vi "ModbusReadHD220.vi"(0 "Modbus master out 3":refnum<class "Modbus Master.lvclass">, 11 "error in (no error)":errorcluster caption="에러 입력(에러 없음)") -> (4 "Modbus master out":refnum<class "Modbus Master.lvclass">, 6 "24105":u16[](array[numeric]), 8 "20600":bool[](array[boolean]), 13 "21600(0)":bool[](array[boolean]), 14 "21600(1)":bool[](array[boolean]), 15 "error out":errorcluster caption="에러 출력")   [LabVIEW 2019]
uses:
  <vilib>/NI/Modbus Library/API/Master/Modbus Master.lvclass
panel:
  out "24019":u16[](array[numeric])
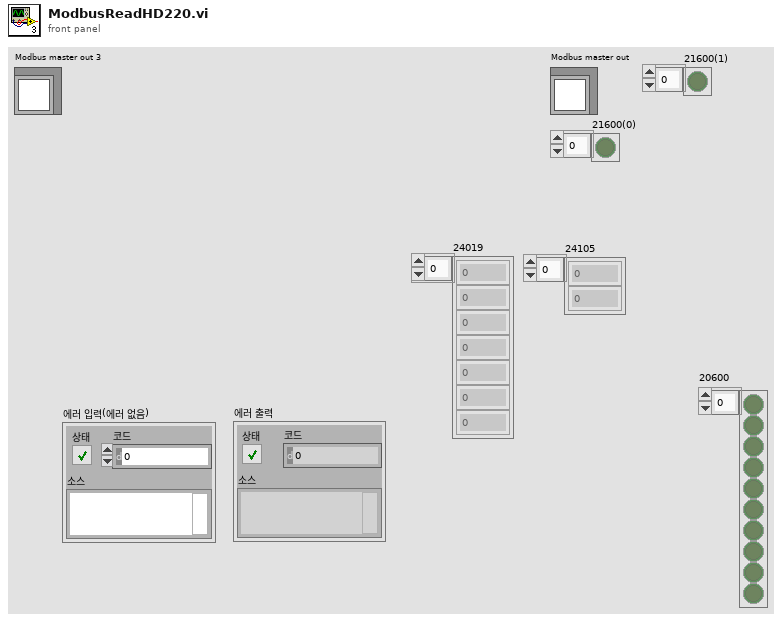
[diagram p1: front panel]
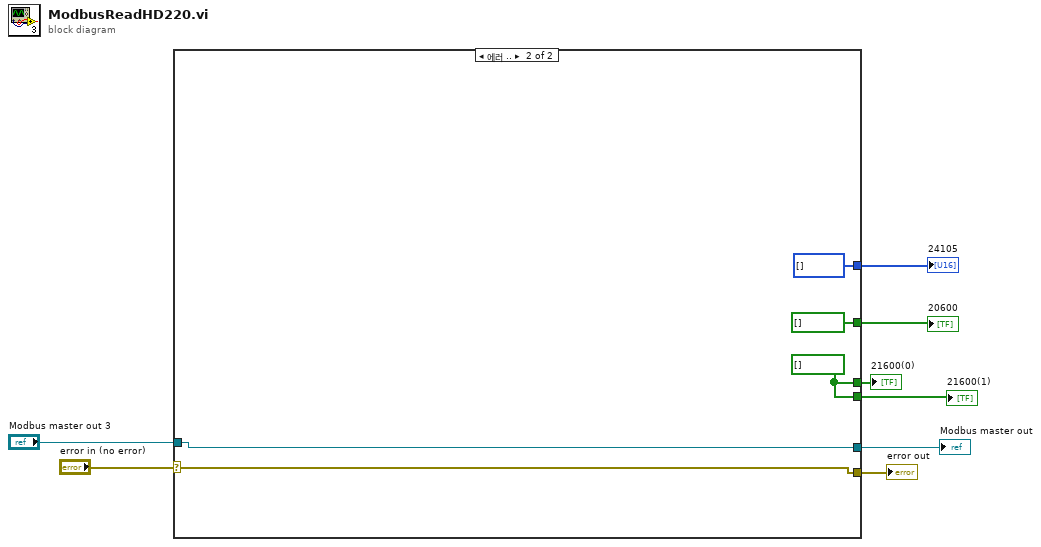
[diagram p0: block diagram]
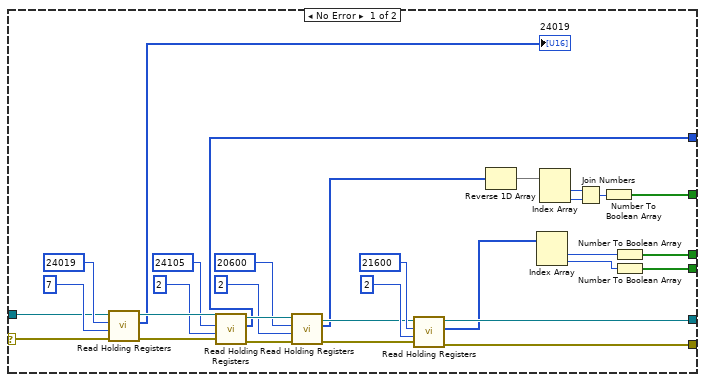
[diagram p2: hidden frame]
diagram:
  n1 = case shown="에러 .." "error in (no error)" {
    selector: "error in (no error)" -> [w37 w43]
    tunnel: "Modbus master out 3" -> [w32 w44]
    tunnel: [w23 w43] -> w6
    tunnel: [w22 w44] -> w5
    tunnel: [w15 bool[] [] ("Boolean array")] -> w4
    tunnel: [w14 u16[] [] ("register values")] -> w3
    tunnel: [w10 w40] -> w1
    tunnel: [w9 w40] -> w2
    frame No Error {
      n2 = call-dynamic "Read Holding Registers.vi"("error in"=w37, "number of inputs"=u16 7, "starting address"=u16 24019, "Modbus master in"=w32) -> ("error out"=w36:errorcluster, "register values"=→"24019":u16[], "Modbus master out"=w35:refnum<class "Modbus Master.lvclass">)  [unwired: 5 in]
      n3 = call-dynamic "Read Holding Registers.vi"("error in"=w36, "number of inputs"=u16 2, "starting address"=u16 24105, "Modbus master in"=w35) -> ("error out"=w33:errorcluster, "register values"=w14:u16[], "Modbus master out"=w34:refnum<class "Modbus Master.lvclass">)  [unwired: 5 in]
      n4 = call-dynamic "Read Holding Registers.vi"("error in"=w33, "number of inputs"=u16 2, "starting address"=u16 20600, "Modbus master in"=w34) -> ("error out"=w25:errorcluster, "register values"=w16:u16[], "Modbus master out"=w24:refnum<class "Modbus Master.lvclass">)  [unwired: 5 in]
      n5 = call-dynamic "Read Holding Registers.vi"("error in"=w25, "number of inputs"=u16 2, "starting address"=u16 21600, "Modbus master in"=w24) -> ("error out"=w23:errorcluster, "register values"=w13:u16[], "Modbus master out"=w22:refnum<class "Modbus Master.lvclass">)  [unwired: 5 in]
      n6 = Reverse 1D Array(array=w16) -> (reversed array=w20:u16[])
      n7 = Index Array(array=w13) -> (element #1=w12:u16, element #2=w11:u16)  [unwired: 2 in]
      n8 = Index Array(array=w20) -> (element #1=w19:u16, element #2=w18:u16)  [unwired: 2 in]
      n9 = Join Numbers(hi=w19, lo=w18) -> ((hi.lo)=w17:u32)
      n10 = Number To Boolean Array(number=w17) -> (Boolean array=w15:bool[])
      n11 = Number To Boolean Array(number=w12) -> (Boolean array=w9:bool[])
      n12 = Number To Boolean Array(number=w11) -> (Boolean array=w10:bool[])
    }
    frame Error {
      w40 = bool[] [] ("Boolean array")
    }
  }
  "error out" <- w6
  "Modbus master out" <- w5
  "20600" <- w4
  "24105" <- w3
  "21600(0)" <- w2
  "21600(1)" <- w1
